vi "input.vi"(8 "error in":errorcluster, 10 "input allocation":T1, 11 "module in":refnum<class "E2E Runtime (UDP).lvclass">) -> (0 "error out":errorcluster, 2 "input data":T1, 3 "module out":refnum<class "E2E Runtime (UDP).lvclass">)   [LabVIEW 2015, in "E2E Runtime (UDP).lvclass"]
doc: "Provides an interface for reading data from a module at runtime. While this interface performs no operations, a child should provide an override which may read from any open sessions, references, or interfaces."
uses:
  E2E Runtime (UDP).lvclass
  <vilib>/NI/Tag Bus/table/data table.ctl
  E2E Runtime (UDP).lvclass/E2E Runtime (UDP).ctl
  <vilib>/NI/Tag Bus/table/data table.lvlib
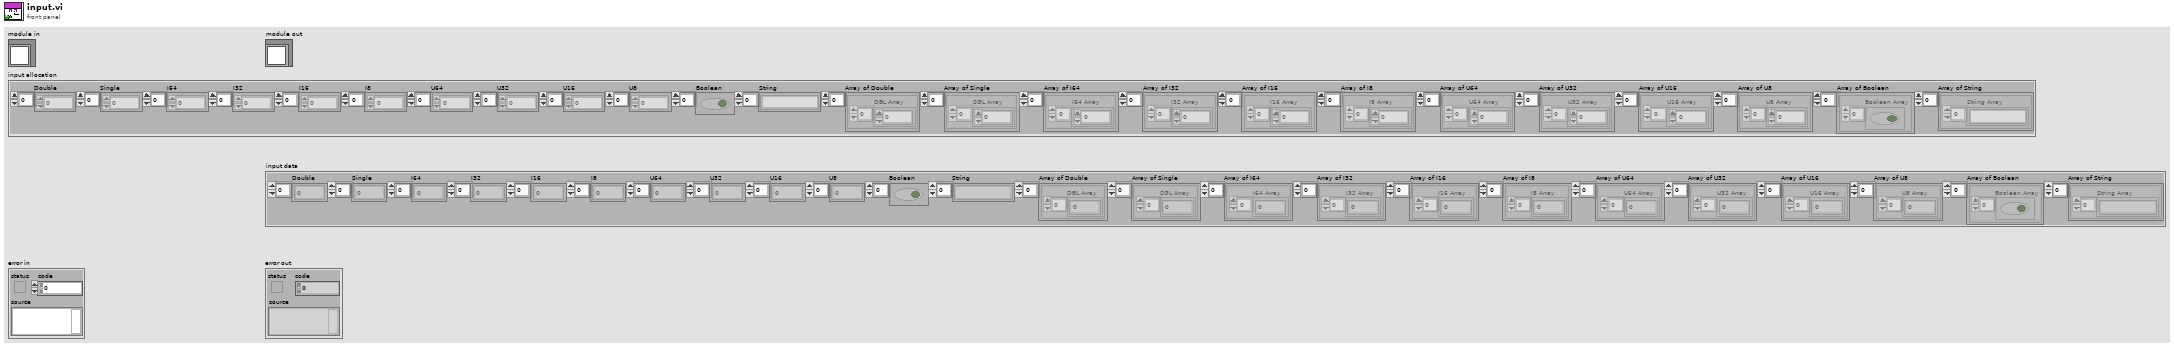
[diagram p1: front panel]
types:
  T1 = typedef "tag bus.lvlib/data table.lvlib/data table.ctl" = cluster{"Double":dbl[], "Single":sgl[], "I64":i64[], "I32":i32[], "I16":i16[], "I8":i8[], "U64":u64[], "U32":u32[], "U16":u16[], "U8":u8[], "Boolean":bool[], "String":string[], "Array of Double":cluster{"DBL Array":dbl[]}[], "Array of Single":cluster{"SGL Array":sgl[]}[], "Array of I64":cluster{"I64 Array":i64[]}[], "Array of I32":cluster{"I32 Array":i32[]}[], "Array of I16":cluster{"I16 Array":i16[]}[], "Array of I8":cluster{"I8 Array":i8[]}[], "Array of U64":cluster{"U64 Array":u64[]}[], "Array of U32":cluster{"U32 Array":u32[]}[], "Array of U16":cluster{"U16 Array":u16[]}[], "Array of U8":cluster{"U8 Array":u8[]}[], "Array of Boolean":cluster{"Boolean Array":bool[]}[], "Array of String":cluster{"String Array":string[]}[]}
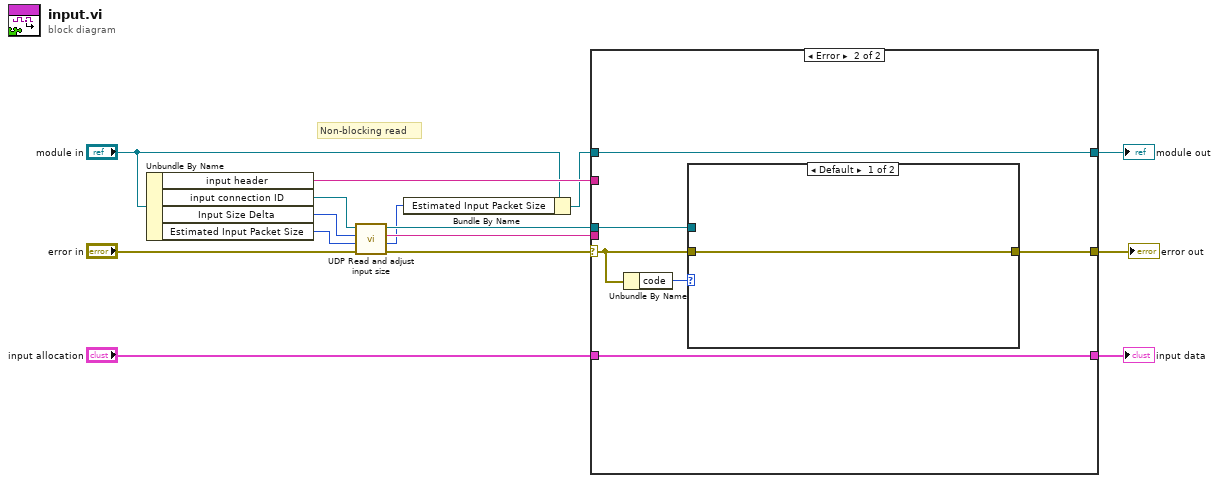
[diagram p0: block diagram]
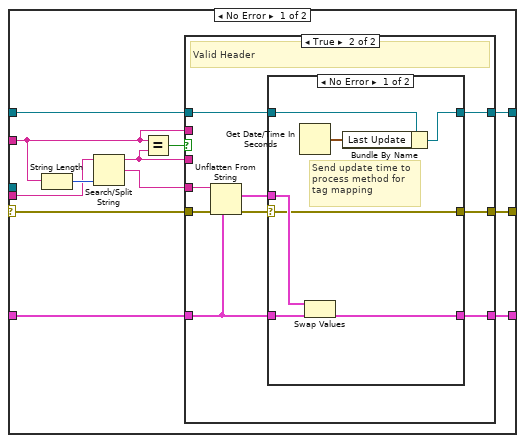
[diagram p2: hidden frame]
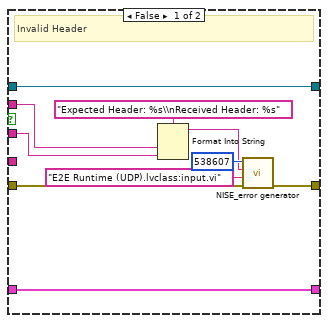
[diagram p3: hidden frame]
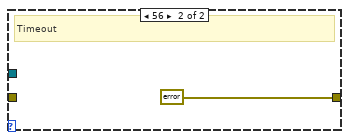
[diagram p5: hidden frame]
diagram:
  # "Non-blocking read"
  n1 = Unbundle By Name("module in") -> ("input header"=w15:string, "input connection ID"=w8:refnum<k16>, "Input Size Delta"=w6:i32, "Estimated Input Packet Size"=w5:i32)
  n2 = call "UDP Read and adjust input size.vi"("error in (no error)"="error in", "Estimated input size"=w5, "Input Size Delta"=w6, "connection ID"=w8) -> ("error out"=w10:errorcluster, "Estimated input size out"=w3:i32, "data out"=w4:string, "connection ID out"=w9:refnum<k16>)  [unwired: 4 in]
  n3 = Bundle By Name(cluster="module in", "Estimated Input Packet Size"=w3) -> (w1:refnum<class "E2E Runtime (UDP).lvclass">)
  n4 = case shown="Error" w10 {
    selector: w10 -> [w24 w62]
    tunnel: [w18 w60] -> w11
    tunnel: w4 -> [w26 _]
    tunnel: w15 -> [w16 _]
    tunnel: "input allocation" -> [w23 w58]
    tunnel: w1 -> [w21 w59]
    tunnel: [w20 w58] -> w13
    tunnel: [w19 w59] -> w12
    tunnel: w9 -> [_ w57]
    frame No Error {
      n5 = String Length(string=w16) -> (length=w27:i32)
      n6 = Search/Split String(string=w26, offset (0)=w27) -> (substring before match=w17:string, match + rest of string=w25:string)  [unwired: 1 in, 1 out]
      n7 = Equal?(x=w16, y=w17) -> (x = y?=w22:bool)
      n8 = case shown="True" w22 {
        tunnel: w25 -> [_ w46]
        tunnel: w24 -> [w35 w45]
        tunnel: w23 -> [w36 w43]
        tunnel: w21 -> [w37 w41]
        tunnel: [w36 w40] -> w20
        tunnel: [w37 w39] -> w19
        tunnel: [w34 w38] -> w18
        tunnel: w17 -> [w29 _]
        tunnel: w16 -> [w30 _]
        frame False {
          # "Invalid Header"
          n9 = Format Into String(format string="Expected Header: %s\\nReceived Header: %s", w30, w29) -> (resulting string=w28:string)  [unwired: 2 in, 1 out]
          n10 = call <vilib>:"NISE_error generator.vi"("error in"=w35, "source"="E2E Runtime (UDP).lvclass:input.vi", "append error message"=w28, "error code (0)"=538607) -> ("error out"=w34:errorcluster)  [unwired: 5 in]
        }
        frame True {
          # "Valid Header"
          n11 = Unflatten From String(type=w43, binary string=w46, error in (no error)=w45) -> (value=w44:T1, error out=w42:errorcluster)  [unwired: 2 in, 1 out]
          n12 = case shown="No Error" w42 {
            selector: w42 -> [w47 w54]
            tunnel: w44 -> [w53 _]
            tunnel: w43 -> [w52 w55]
            tunnel: w41 -> [w51 w56]
            tunnel: [w49 w55] -> w40
            tunnel: [w48 w56] -> w39
            tunnel: [w47 w54] -> w38
            frame No Error {
              # "Send update time to\nprocess method for\ntag mapping"
              n13 = Get Date/Time In Seconds() -> (seconds since 1Jan1904=w50:timestamp)
              n14 = Swap Values(12:w53, 14:w52) -> (3:w49:T1)  [unwired: 1 in, 1 out]
              n15 = Bundle By Name(cluster=w51, "Last Update"=w50) -> (w48:refnum<class "E2E Runtime (UDP).lvclass">)
            }
            frame Error {
            }
          }
        }
      }
    }
    frame Error {
      n16 = Unbundle By Name(w62) -> ("code"=w61:i32)
      n17 = case shown="Default" w61 {
        tunnel: w62 -> [w63 _]
        tunnel: [w63 errorcluster {"status"=FALSE, "code"=0, "source"=""} ("error IO")] -> w60
        tunnel: w57 -> [_ _]
        frame Default {
        }
        frame 56 {
          # "Timeout"
        }
      }
    }
  }
  "error out" <- w11
  "module out" <- w12
  "input data" <- w13
